vi "camera system compressed.vi"() -> (0 "ball or wrong size cube 2":bool, 1 "pink":bool, 2 "yellow":bool, 3 "blue":bool, 4 "big, mid, small":string)   [LabVIEW 2026]
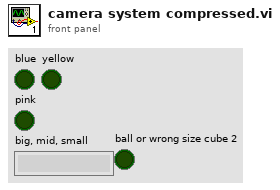
[diagram p1: front panel]
types:
  T1 = typedef "IMAQ Image.ctl" = refnum<image>
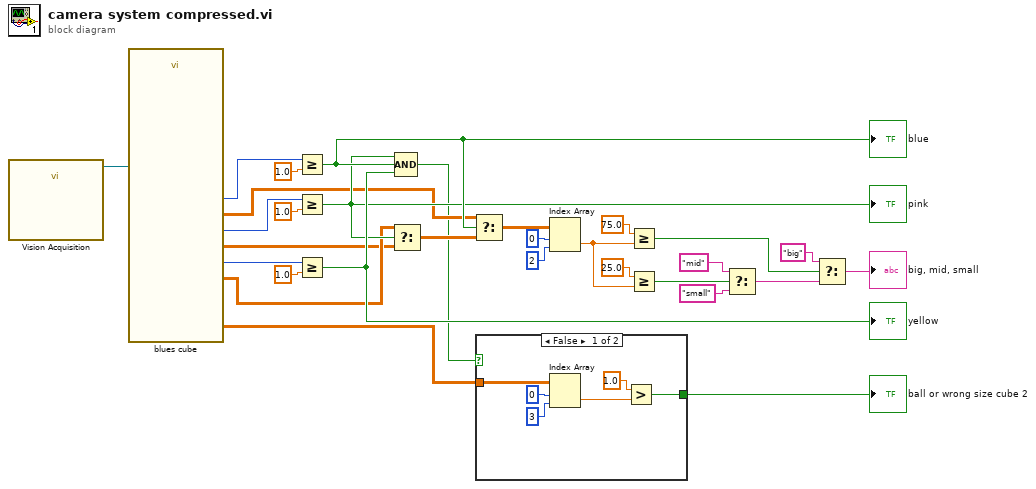
[diagram p0: block diagram]
diagram:
  n1 = call "Vision Acquisition"() -> ("Image Out"=w30:T1)  [unwired: 26 in, 1 out]
  n2 = call "blues cube"("Image In"=w30) -> ("Particle Measurements (Pixels) (Particle Analysis 4)"=w1:dbl[][], "Number of Particles (Particle Analysis 1)"=w11:i32, "Particle Measurements (Pixels) (Particle Analysis 1)"=w8:dbl[][], "Number of Particles (Particle Analysis 3)"=w10:i32, "Particle Measurements (Pixels) (Particle Analysis 3)"=w7:dbl[][], "Number of Particles (Particle Analysis 2)"=w5:i32, "Particle Measurements (Pixels) (Particle Analysis 2)"=w4:dbl[][])  [unwired: 17 in, 3 out]
  n3 = Greater Or Equal?(x=w11, y=1.0) -> (x >= y?=w29:bool)
  "blue" <- w29
  n4 = Greater Or Equal?(x=w5, y=1.0) -> (x >= y?=w26:bool)
  "pink" <- w26
  n5 = Greater Or Equal?(x=w10, y=1.0) -> (x >= y?=w28:bool)
  "yellow" <- w28
  n6 = Select(t=w7, s=w26, f=w4) -> (s? t:f=w27:dbl[][])
  n7 = Compound Arithmetic op=AND(w26, w29, w28) -> (w2:bool)
  n8 = Select(t=w8, s=w29, f=w27) -> (s? t:f=w9:dbl[][])
  n9 = case shown="False" w2 {
    tunnel: [w32 _] -> w3
    tunnel: w1 -> [w31 _]
    frame False {
      n10 = Index Array(array=w31, index (row)=0, index (col)=3 ("Numeric")) -> (element=w33:dbl)
      n11 = Greater?(x=1.0, y=w33) -> (0:w32:bool)
    }
    frame True {
    }
  }
  "ball or wrong size cube 2" <- w3
  n12 = Index Array(array=w9, index (row)=0, index (col)=2 ("disabled index (col)")) -> (element=w6:dbl)
  n13 = Greater Or Equal?(x=75.0, y=w6) -> (x >= y?=w20:bool)
  n14 = Greater Or Equal?(x=25.0, y=w6) -> (x >= y?=w21:bool)
  n15 = Select(t="mid", s=w21, f="small") -> (s? t:f=w22:string)
  n16 = Select(t="big", s=w20, f=w22) -> (s? t:f=→"big, mid, small":string)
